vi "VIH HelpGen - Open VI Reference (Basic).vi"(6 "Without Refees (F)":bool, 8 "error in":errorcluster, 9 "options":i32 format="%.0x", 11 "VI Path":path) -> (0 "error out":errorcluster, 3 "VI Reference":refnum<vi>, 5 "Tmp App Refnum":refnum<vi>)   [LabVIEW 2014]
doc: "::: VI Helpeks :::\nCopyright (c) 2000-2026 Konstantin Shifershteyn. All rights reserved."
panel:
  # "VI Helpeks\nCopyright (c) 2012-2026 Konstantin Shifershteyn"
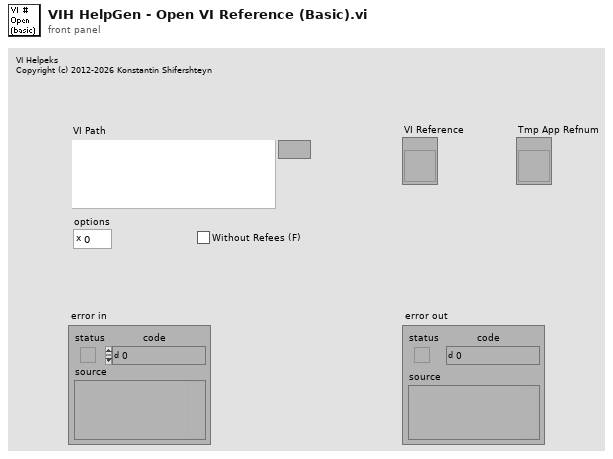
[diagram p1: front panel]
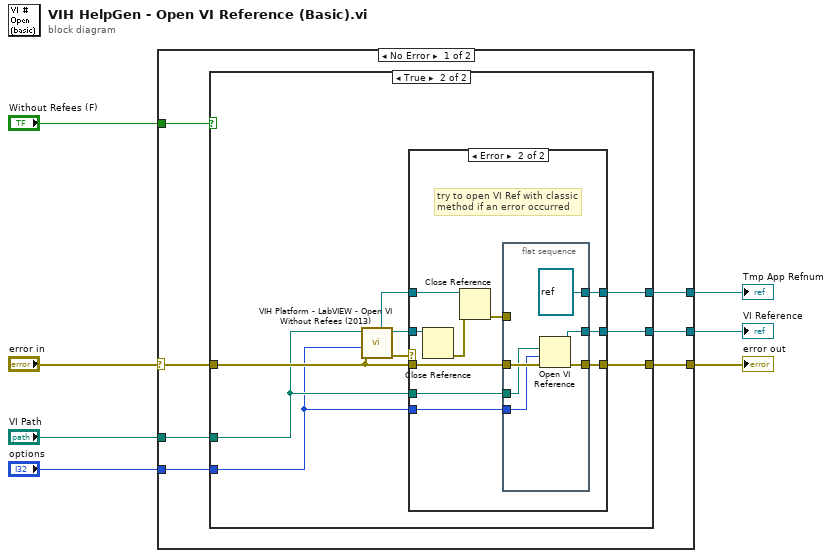
[diagram p0: block diagram]
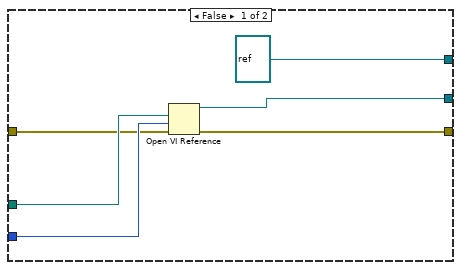
[diagram p2: hidden frame]
diagram:
  n1 = case shown="No Error" "error in" {
    selector: "error in" -> [w8 w49]
    tunnel: "options" -> [w14 _]
    tunnel: "VI Path" -> [w13 _]
    tunnel: [w12 w49] -> w5
    tunnel: [w11 _] -> w4
    tunnel: [w10 _] -> w3
    tunnel: "Without Refees (F)" -> [w9 _]
    frame No Error {
      n2 = case shown="True" w9 {
        tunnel: w14 -> [w20 w21]
        tunnel: w13 -> [w19 w22]
        tunnel: w8 -> [w18 w23]
        tunnel: [w17 w27] -> w12
        tunnel: [w16 w28] -> w11
        tunnel: [refnum<vi> refnum ("App Refnum") w29] -> w10
        frame False {
          n3 = Open VI Reference(vi path=w19, options=w20, error in (no error)=w18) -> (vi reference=w16:refnum<vi>, error out=w17:errorcluster)  [unwired: 3 in]
        }
        frame True {
          n4 = call "VIH Platform - LabVIEW - Open VI Without Refees (2013).vi"("error in"=w23, "options"=w21, "VI Path"=w22) -> ("error out"=w24:errorcluster, "VI Reference"=w26:refnum<vi>, "Tmp App Refnum"=w25:refnum<vi>)  [unwired: 6 in]
          n5 = case shown="Error" w24 {
            selector: w24 -> [w30 _]
            tunnel: w25 -> [w32 w38]
            tunnel: [w32 w40] -> w29
            tunnel: w26 -> [w31 w39]
            tunnel: [w31 w41] -> w28
            tunnel: [w30 w42] -> w27
            tunnel: w23 -> [_ w36]
            tunnel: w22 -> [_ w35]
            tunnel: w21 -> [_ w34]
            frame No Error {
            }
            frame Error {
              # "try to open VI Ref with classic\nmethod if an error occurred"
              n6 = Close Reference(reference=w39) -> (error out=w37:errorcluster)  [unwired: 1 in]
              n7 = Close Reference(reference=w38, error in (no error)=w37) -> (error out=w33:errorcluster)
              n8 = flat-sequence {
                tunnel: [w48] -> w42
                tunnel: [w47] -> w41
                tunnel: [refnum<vi> refnum ("App Refnum")] -> w40
                tunnel: w36 -> [w45]
                tunnel: w35 -> [w44]
                tunnel: w34 -> [w43]
                tunnel: w33 -> [_]
                frame #0 {
                  n9 = Open VI Reference(vi path=w44, options=w43, error in (no error)=w45) -> (vi reference=w47:refnum<vi>, error out=w48:errorcluster)  [unwired: 3 in]
                }
              }
            }
          }
        }
      }
    }
    frame Error {
    }
  }
  "VI Reference" <- w4
  "error out" <- w5
  "Tmp App Refnum" <- w3
